vi "Grid_Create.vi"(0 "reference":refnum<class "Grid.lvclass">, 1 "gridColor":u32(colorbox), 5 "error in (no error)":errorcluster) -> (14 "reference out":refnum<class "Grid.lvclass">, 16 "# of objects":i32, 19 "error out":errorcluster)   [LabVIEW 2020, in "Grid.lvclass"]
doc: "Creates and initializes a new Grid object.\n\nThis object should be destroyed using a Grid destructor VI.\n\n[GOOP 2.1]"
uses:
  <resource>/Framework/Providers/Open_GDS/UML/Grid_class/Grid.lvclass
panel:
  # "The input reference should only\nbe wired when this method is called\nby a sub class constructor."
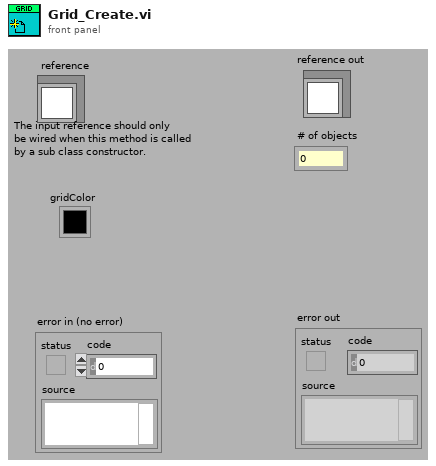
[diagram p1: front panel]
types:
  T1 = typedef "Grid.lvclass/ObjectAttributes.ctl" = cluster{"gridX":dbl, "gridY":dbl, "gridColor":u32}
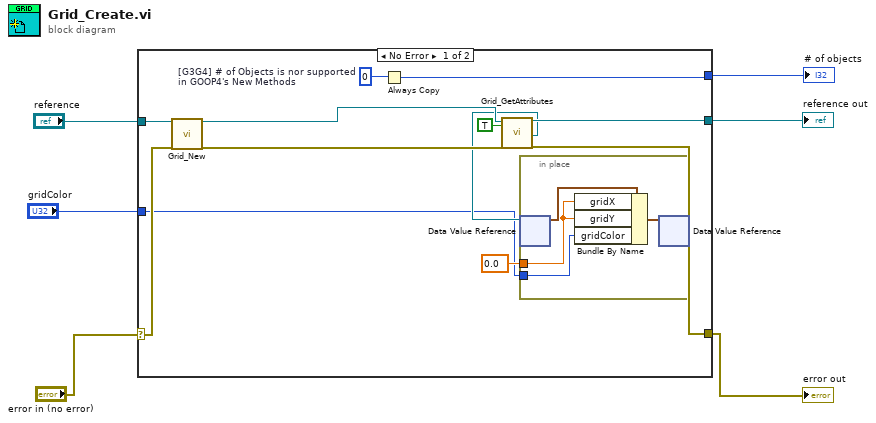
[diagram p0: block diagram]
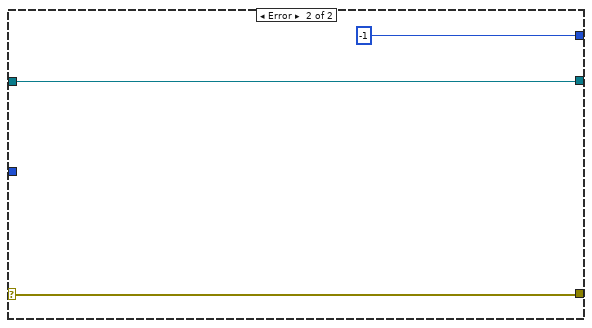
[diagram p2: hidden frame]
diagram:
  n1 = case shown="No Error" "error in (no error)" {
    selector: "error in (no error)" -> [w18 w24]
    tunnel: [w16 w23] -> w6
    tunnel: [w17 w24] -> w5
    tunnel: [w12 -1 ("Nr of open handles")] -> w4
    tunnel: "reference" -> [w15 w23]
    tunnel: "gridColor" -> [w8 _]
    frame No Error {
      w7 = 0  # [G3G4] # of Objects is nor supported in GOOP4's New Methods
      n2 = call <resource>:"Grid_New.vi"("reference in"=w15, "error in (no error)"=w18) -> ("reference out"=w14:refnum<class "Grid.lvclass">, "error out"=w13:errorcluster)  [unwired: 3 in, 13 out]
      n3 = Always Copy(1:w7) -> (0:w12:i32)
      n4 = call <resource>:"Grid_GetAttributes.vi"("reference in"=w14, "OnlyGetDvrReference(False)"=TRUE, "error in (no error)"=w13) -> ("reference out"=w16:refnum<class "Grid.lvclass">, "DataRef"=w10:refnum<data-value>, "error out"=w17:errorcluster)  [unwired: 13 in, 1 out]
      n5 = in-place {
        in-place-border: 0.0 ("gridX") -> [w21]
        in-place-border: w8 -> [w20]
        n6 = in-place-dvr #1(w10) -> (w22:T1)  [unwired: 1 out]
        n7 = Bundle By Name(cluster=w22, "gridX"=w21, "gridY"=w21, "gridColor"=w20) -> (w19:T1)
        n8 = in-place-dvr #1(w19) -> ()  [unwired: 2 out]
      }
    }
    frame Error {
    }
  }
  "error out" <- w5
  "reference out" <- w6
  "# of objects" <- w4
